vi "Native_AddWhile_v3.vi"() -> ()   [LabVIEW 2024]
uses:
  <vilib>/Utility/miscctls.llb/LVBoundsTypeDef.ctl
panel:
  out "error out":errorcluster caption="错误输出"
  out "loop_id":u32
  in  "loop_id type":u32
  in  "bounds":T1 caption="边界"
  in  "y":i16=100
  in  "x":i16=100
  in  "style":u32
  in  "owner_diagram_id":u32
  in  "target_path":path
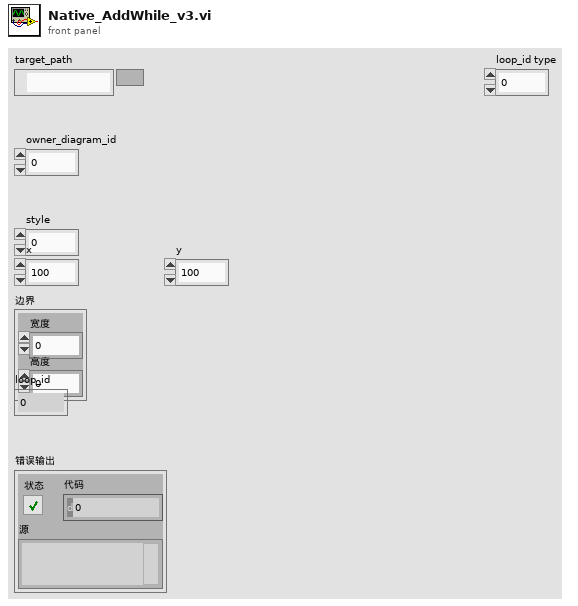
[diagram p1: front panel]
types:
  T1 = typedef "LVBoundsTypeDef.ctl" = cluster{"Width":u32, "Height":u32}
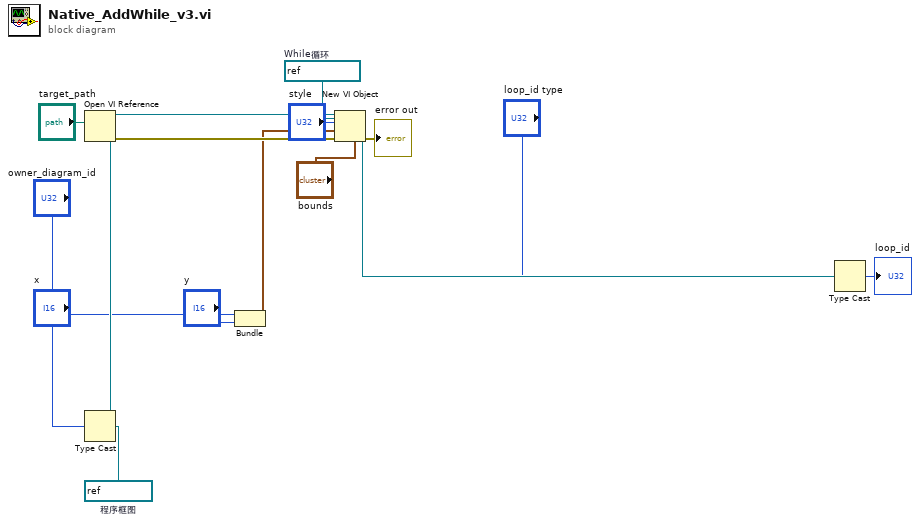
[diagram p0: block diagram]
diagram:
  w12 = refnum<vi> refnum  # While循环
  w13 = refnum<vi> refnum  # 程序框图
  n1 = Open VI Reference ("打开VI引用")(vi path="target_path") -> (error out=w10:errorcluster)  [unwired: 5 in, 1 out]
  n2 = Type Cast ("强制类型转换")(type=w13, x="owner_diagram_id") -> (*(type *) &x=w11:refnum<vi>)
  n3 = Bundle ("捆绑")("x"="x", "y"="y") -> (w6:cluster{"x":i16, "y":i16})  [unwired: 1 in]
  n4 = New VI Object ("新建VI对象")(vi object class=w12, owner refnum=w11, style="style", position/next to=w6, 4:"bounds", 8:w10) -> (object refnum=w4:refnum<vi>, 0:→"error out":errorcluster)  [unwired: 2 in]
  n5 = Type Cast ("强制类型转换")(type="loop_id type", x=w4) -> (*(type *) &x=→"loop_id":u32)
